vi "Measurement Logic.vi"(8 "error in":errorcluster, 9 "measurement configuration":T2={"INTERFACE NAME STRING"="Lorem ipsum dolor sit", "Payload"="", "Protocol Layer 2"={"Has VLAN"=FALSE, "VLAN TAG"={"TPID"=0, "PRIORITY"=0, "DEI"=FALSE, "VID"=0}, "DESTINATION MAC ADDRESS"="", "ETHERTYPE"=0}, "SEND FRAME"=TRUE, "CYCLE?"=FALSE}, 10 "measure call context in":refnum<class "Measure Call Context.lvclass">, 11 "user event out":refnum<user-event>) -> (0 "error out":errorcluster, 1 "measurement results":T1={"Transmitting"=FALSE, "RECEIVED PACKETS"=0, "STATUS"="Empty", "OOB gRPC Port"=0}, 2 "measure call context out":refnum<class "Measure Call Context.lvclass">)   [LabVIEW 2025, in "Automotive Ethernet Frame Generator.lvclass"]
doc: "Contains the core logic for executing the measurement."
uses:
  Automotive Ethernet Frame Generator.lvclass
  Automotive Ethernet Frame Generator.lvclass/Automotive Ethernet Frame Generator.ctl
  <vilib>/Plug-In SDKs/Measurements/Measure Call Context/Measure Call Context.lvclass
  Measurement Results.ctl
  OOB Data Transfer/OOB Data Transfer.lvlib
  <vilib>/xnet/xnet.llb/XNET Create Session (Frame Output Stream).vi
  <vilib>/xnet/xnet.llb/XNET Write (Frame Ethernet).vi
  Measurement Configuration.ctl
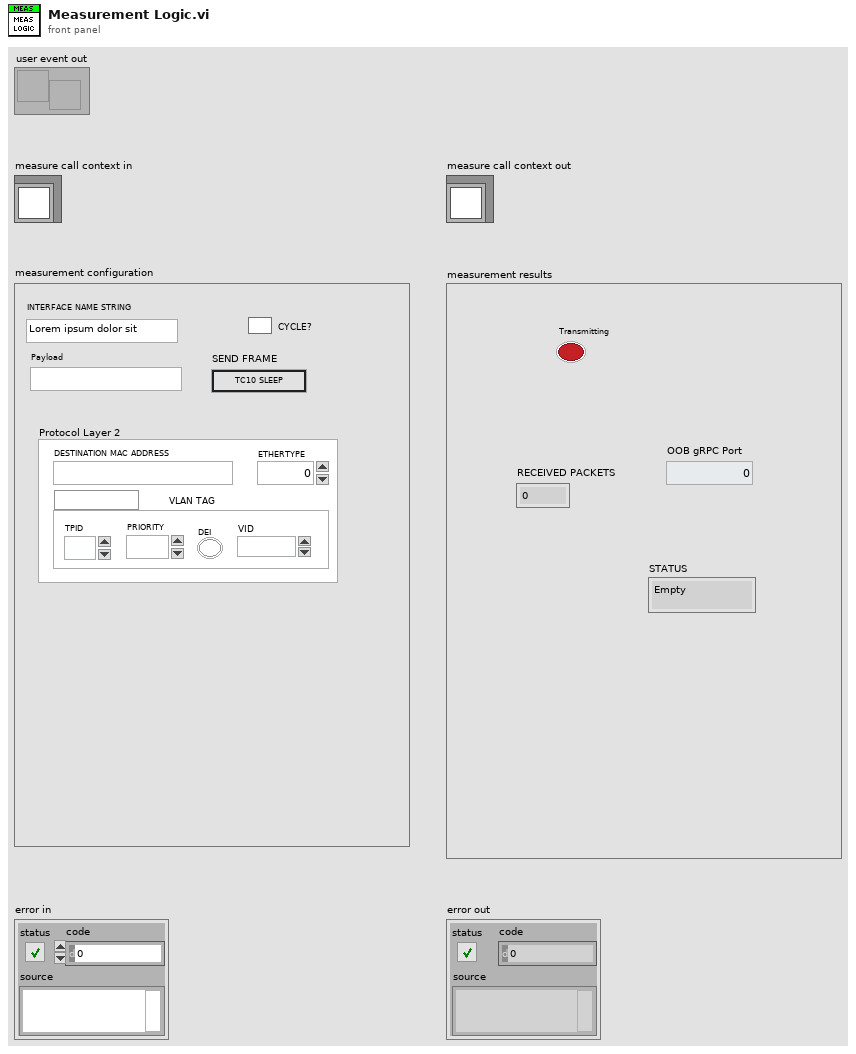
[diagram p1: front panel]
types:
  T1 = typedef "Automotive Ethernet Frame Generator.lvclass/Measurement Results.ctl" = cluster{"Transmitting":bool, "RECEIVED PACKETS":i32, "STATUS":string, "OOB gRPC Port":i32}
  T2 = typedef "Automotive Ethernet Frame Generator.lvclass/Measurement Configuration.ctl" = cluster{"INTERFACE NAME STRING":string, "Payload":string, "Protocol Layer 2":cluster{"Has VLAN":bool, "VLAN TAG":cluster{"TPID":u16, "PRIORITY":u8, "DEI":bool, "VID":u16}, "DESTINATION MAC ADDRESS":string, "ETHERTYPE":u16}, "SEND FRAME":bool, "CYCLE?":bool}
  T3 = typedef "OOB Data Transfer.lvlib/OOB to Logic Data.ctl" = cluster{"CYCLE":bool, "INTERFACE NAME STRING":string, "PAYLOAD":string, "Protocol Layer":cluster{"Has VLAN":bool, "VLAN TAG":cluster{"TPID":u16, "PRIORITY":u8, "DEI":bool, "VID":u16}, "DESTINATION MAC ADDRESS":string, "ETHERTYPE":u16}, "SEND FRAME":bool}
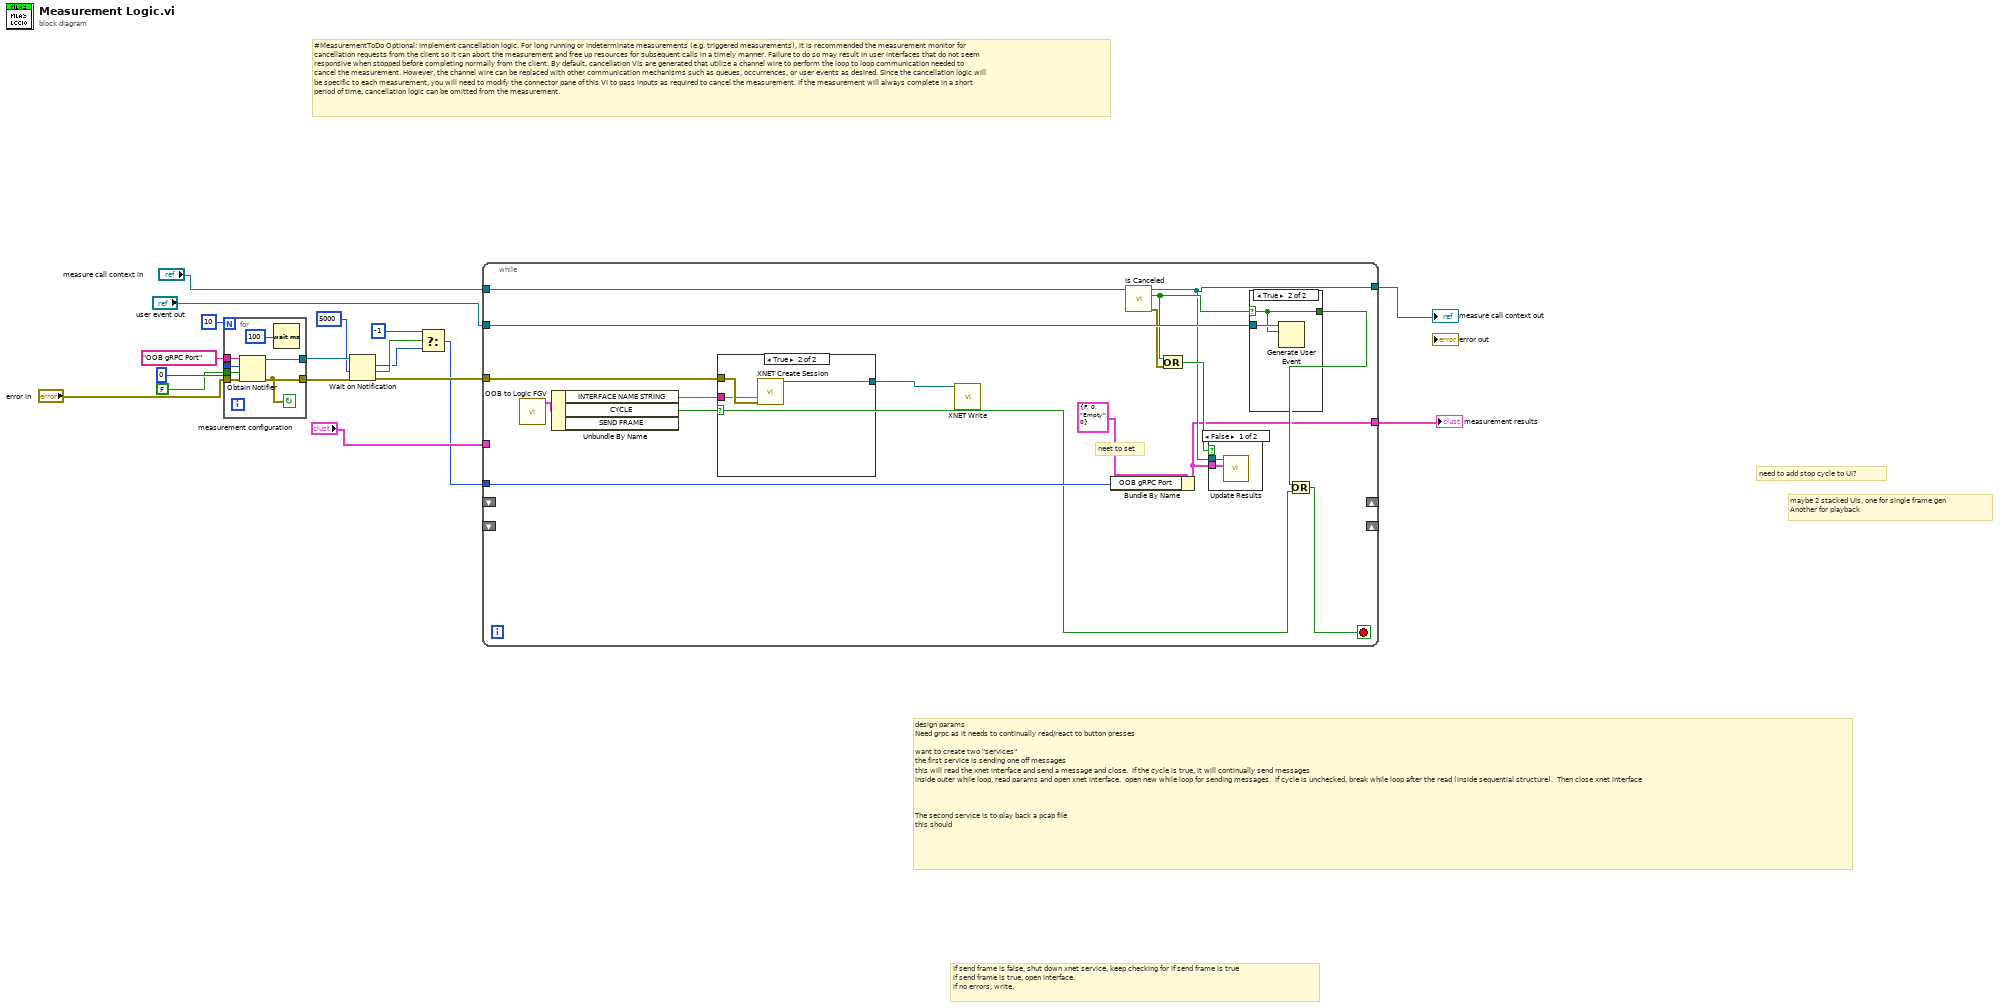
[diagram p0: block diagram]
diagram:
  # "if send frame is false, shut down xnet service, keep checking for if send frame is true\nif send frame is true, open interface.  \nif no errors, write,"
  # "maybe 2 stacked UIs, one for single frame gen\nAnother for playback"
  # "need to add stop cycle to UI?"
  # "design params\nNeed grpc as it needs to continually read/react to button presses\n\nwant to create two \"services\"\nthe first service is sending one off messages\nthis will read the xnet interface and send a message and close.  If the cycle is true, it will continually send messages\ninside outer while loop, read params and open xnet interface.  open new while loop for sending messages.  If cycle is unchecked, break while loop after the read (inside sequential structure).  Then close xnet interface\n\n\n\nThe second service is to play back a pcap file\nthis should"
  # "#MeasurementToDo Optional: Implement cancellation logic. For long running or indeterminate measurements (e.g. triggered measurements), it is recommended the measurement monitor for cancellation requests from the client so it can abort the measurement and free up resources for subsequent calls in a timely manner. Failure to do so may result in user interfaces that do not seem responsive when stopped before completing normally from the client. By default, cancellation VIs are generated that utilize a channel wire to perform the loop to loop communication needed to cancel the measurement. However, the channel wire can be replaced with other communication mechanisms such as queues, occurrences, or user events as desired. Since the cancellation logic will be specific to each measurement, you will need to modify the connector pane of this VI to pass inputs as required to cancel the measurement. If the measurement will always complete in a short period of time, cancellation logic can be omitted from the measurement."
  n1 = for {
    N: 10 -> [_]
    tunnel: [w23] -> w13
    tunnel: [w25] -> w9
    tunnel: "OOB gRPC Port" ("name") -> [w22]
    tunnel: 0 ("i32") -> [w21]
    tunnel: "error in" -> [w20]
    tunnel: FALSE ("create if not found?") -> [w19]
    stop <- w23 continue-if-true
    n2 = Obtain Notifier(name (unnamed)=w22, notification data type=w21, create if not found? (T)=w19, error in (no error)=w20) -> (notifier out=w25:refnum<notifier>, error out=w23:errorcluster)  [unwired: 1 out]
    n3 = Wait (ms)(milliseconds to wait=u32 100) -> ()  [unwired: 1 out]
  }
  n4 = Wait on Notification(notifier=w9, timeout in ms (-1)=5000, error in (no error)=w13) -> (notification=w11:i32, timed out?=w12:bool, error out=w7:errorcluster)  [unwired: 1 in, 1 out]
  n5 = Select(t=-1, s=w12, f=w11) -> (s? t:f=w1:i32)
  n6 = while {
    tunnel: "measurement configuration" -> [_]
    tunnel: w7 -> [w41]
    tunnel: "user event out" -> [w39]
    tunnel: "measure call context in" -> [w33]
    tunnel: [w31] -> w2
    tunnel: [w32] -> w3
    tunnel: w1 -> [w29]
    shift-right: _ -> [_]
    shift-left: _ -> [_]
    shift-right: _ -> [_]
    shift-left: _ -> [_]
    stop <- w37 stop-if-true
    # "neet to set"
    n7 = call "OOB to Logic FGV.vi"() -> ("OOB to Logic Data out"=w28:T3)  [unwired: 10 in, 1 out]
    n8 = Unbundle By Name(w28) -> ("INTERFACE NAME STRING"=w40:string, "CYCLE"=w27:bool)  [unwired: 1 out]
    n9 = case shown="True" {
      selector: _ -> [_ _]
      tunnel: w41 -> [_ w44]
      tunnel: w40 -> [_ w43]
      tunnel: [_ w42] -> w26
      frame False {
      }
      frame True {
        n10 = call-poly <vilib>:"XNET Create Session.vi"("interface"=w43, "error in (no error)"=w44) -> ("session out"=w42:refnum<k21>)  [unwired: 12 in, 1 out]
      }
    }
    n11 = call-poly <vilib>:"XNET Write.vi"("session in"=w26) -> ()  [unwired: 13 in, 2 out]
    n12 = Bundle By Name(cluster=T1 {"Transmitting"=FALSE, "RECEIVED PACKETS"=0, "STATUS"="Empty", "OOB gRPC Port"=0} ("measurement results 2"), "OOB gRPC Port"=w29) -> (w31:T1)
    n13 = call <vilib>:"Is Canceled.vi"("measure call context in"=w33) -> ("error out"=w35:errorcluster, "is canceled?"=w36:bool, "measure call context out"=w32:refnum<class "Measure Call Context.lvclass">)  [unwired: 8 in]
    n14 = Compound Arithmetic op=OR(w36, w35) -> (w34:bool)
    n15 = case shown="False" w34 {
      tunnel: w32 -> [w46 _]
      tunnel: w31 -> [w45 _]
      frame False {
        n16 = call <vilib>:"Update Results.vi"("measurement results"=w45, "measure call context in"=w46) -> ()  [unwired: 8 in, 2 out]
      }
      frame True {
      }
    }
    n17 = case shown="True" w36 {
      selector: w36 -> [w47 w48]
      tunnel: w39 -> [_ w49]
      tunnel: [w47 w48] -> w38
      frame False {
      }
      frame True {
        n18 = Generate User Event(user event=w49, event data cluster=w48) -> ()  [unwired: 2 in, 2 out]
      }
    }
    n19 = Or(x=w38, y=w27) -> (x .or. y?=w37:bool)
  }
  "measure call context out" <- w3
  "measurement results" <- w2
